vi "P10_VIsInMemory.vi"(11 "Inputs":string[](array[string])) -> (2 "Output/Failure":string, 3 "CLI Process Return Code":i32)   [LabVIEW 2026]
doc: "Slice 1.1 probe: Reads Application All VIs In Memory and searches it for the name in Inputs[0]. Opens no VI by path."
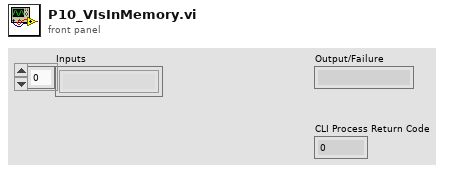
[diagram p1: front panel]
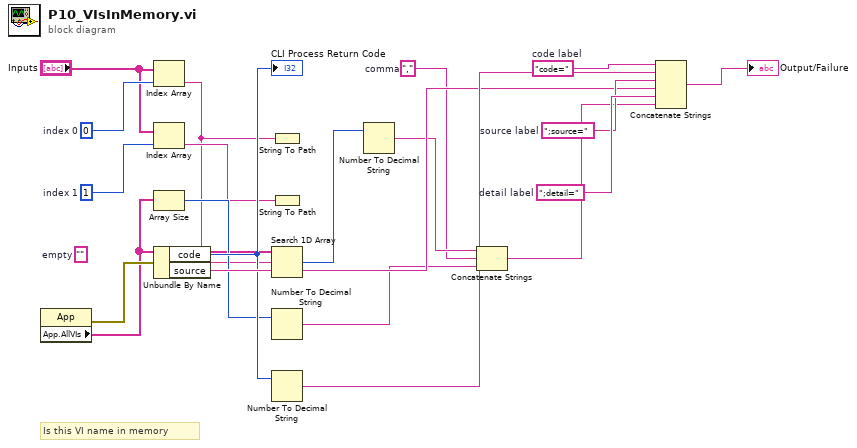
[diagram p0: block diagram]
diagram:
  w19 = ";detail="  # detail label
  w18 = ";source="  # source label
  w17 = "code="  # code label
  w10 = ","  # comma
  (unwired) ""  # empty
  w3 = 1  # index 1
  w2 = 0  # index 0
  # "Is this VI name in memory"
  n1 = property class="App"() -> (error out=w7:errorcluster, "App.AllVIs"=w6:string[])  [unwired: 2 in, 1 out]
  n2 = Index Array(array="Inputs", index=w2) -> (element=w4:string)
  n3 = Index Array(array="Inputs", index=w3) -> (element=w5:string)
  n4 = Array Size(array=w6) -> (size(s)=w9:i32)
  n5 = Unbundle By Name(w7) -> ("code"=w14:i32, "source"=w15:string)
  "CLI Process Return Code" <- w14
  n6 = String To Path(string=w4) -> ()  [unwired: 1 out]
  n7 = String To Path(string=w5) -> ()  [unwired: 1 out]
  n8 = Search 1D Array(1D array=w6, element=w4) -> (index of element=w8:i32)  [unwired: 1 in]
  n9 = Number To Decimal String(number=w9) -> (decimal integer string=w12:string)  [unwired: 1 in]
  n10 = Number To Decimal String(number=w14) -> (decimal integer string=w16:string)  [unwired: 1 in]
  n11 = Number To Decimal String(number=w8) -> (decimal integer string=w11:string)  [unwired: 1 in]
  n12 = Concatenate Strings(w11, w10, w12) -> (w13:string)
  n13 = Concatenate Strings(w17, w16, w18, w15, w19, w13) -> (→"Output/Failure":string)
